vi "lab10.vi"() -> ()   [LabVIEW 2025]
uses:
  vi/thresholds.ctl
  vi/fpga_states.ctl
  <vilib>/rvi/Emulation/niFpgaGetClockAttributes.vi
  <vilib>/rvi/Emulation/niFpgaSctlEmulationGetInTimedLoop.vi
  <vilib>/rvi/Emulation/niFpgaEmulationReportErrorSimple.vi
  <vilib>/rvi/Emulation/niFpgaEmulationIsFPGAContextNoSignature.vi
  <vilib>/rvi/errors/niFpgaSetErrorForExecOnDevCompSimple.vi
  <vilib>/rvi/eio/common/nirviEmuReportErrorAndStop.vi
  <vilib>/rvi/DataTransferAndStorage/Container/Common/niFpgaContainerGetUniqueNameForEmu.vi
  <vilib>/rvi/FIFO/Fifo_Resource/nirvififoEmulationSetSize.vi
  <vilib>/rvi/FIFO/Fifo_Resource/nirviFifoEmulationQueueMgr.vi
  <instcachedir>/0/nirviFifoEmulationQueueMgr_E5CAEC123FF24DC58D834DCA3CDAA9B5.lvgen/nirviFifoEmulationQueueMgr_E5CAEC123FF24DC58D834DCA3CDAA9B5_002.vi
  <vilib>/Utility/error.llb/Clear Errors.vi
  <vilib>/rvi/FIFO/Fifo_Resource/nirvififoEmulationCreateLock.vi
  <vilib>/rvi/Emulation/niFpgaProcessEmulError.vi
  <vilib>/rvi/FIFO/Fifo_Resource/nirvififoEmulationObtainLock.vi
  <vilib>/rvi/FIFO/Fifo_Resource/nirvififoEmulationReleaseLock.vi
  <vilib>/rvi/occurrence/nirviWaitOnOccurrenceBase.vi
  <vilib>/rvi/errors/nirviReportUnexpectedCaseInternalError.vi
  <vilib>/rvi/errors/nirviReportUnexpectedCaseInternalError (U32).vi
  <vilib>/eio/utilities/niEioResolveVilibRelativePath.vi
  <vilib>/rvi/interface/RandomDataEmulation/niFpgaRandomDataHandleErrors.vi
  <vilib>/rvi/Emulation/niFpgaCriticalErrorInLSC.vi
  <instcachedir>/0/nirviFifoEmulationQueueMgr_E5CAEC123FF24DC58D834DCA3CDAA9B5.lvgen/nirviFifoEmulationQueueMgr_E5CAEC123FF24DC58D834DCA3CDAA9B5_003.vi
  <vilib>/rvi/FIFO/Fifo_Resource/nirvififoEmulationDetermineInputValidOut.vi
  <vilib>/rvi/eio/common/nirviEmuTemplateMethod_errors.vi
  <vilib>/rvi/Memory/Memory_Emulation/nirvimemoryFastEmulation.vi
  <vilib>/rvi/Memory/Memory_Emulation/nirvimemoryEmulation.vi
  <vilib>/rvi/DataTransferAndStorage/Container/Common/niFpgaContainerExecOnDevCompGetState.vi
  <vilib>/rvi/Memory/Memory_Emulation/niFpgaMemoryEmulationCacheClearOnFirstRun.vi
  <vilib>/rvi/Memory/Memory_Emulation/nirvimemoryEmulationManagerCache_MakeExclusive.vi
  <vilib>/rvi/Memory/Memory_Emulation/niFpgaMemoryEmulationValidateCache.vi
  <vilib>/rvi/Memory/Memory_Emulation/nirvimemoryEmulationManagerCache_InsertValue.vi
  <vilib>/rvi/Memory/Memory_Emulation/nirvimemoryEmulationManagerCache_ReleaseExclusive.vi
  <vilib>/rvi/Memory/Memory_Emulation/nirvimemoryEmulationManagerCache_GetValue.vi
  <vilib>/rvi/Memory/Memory_Emulation/nirvimemoryEmulationManagerCache_SetValue.vi
  <vilib>/rvi/Emulation/niFpgaSctlEmulationResourceMgr.vi
  <vilib>/rvi/DataTransferAndStorage/Container/XNode/niFpgaContainer.xnode
  <vilib>/rvi/FIFO/Fifo_Resource/nirvififoEmulationRead.vi
  <vilib>/rvi/interface/RandomDataEmulation/nirviRandomDataFpgaReadWriteTemplate.vi
  <vilib>/rvi/FIFO/Fifo_Resource/nirvififoEmulationWrite.vi
  <vilib>/eio/EIONode/EIONode.xnode
  <vilib>/rvi/Memory/Memory_Emulation/niFpgaMemoryEmulationRefIn.vi
panel:
  in  "Threshold":T1
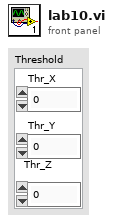
[diagram p1: front panel]
types:
  T1 = typedef "thresholds.ctl" = cluster{"Thr_X":i16, "Thr_Y":i16, "Thr_Z":i16}
  T2 = typedef "fpga_states.ctl" = enum16{"Wait", "Collect"}
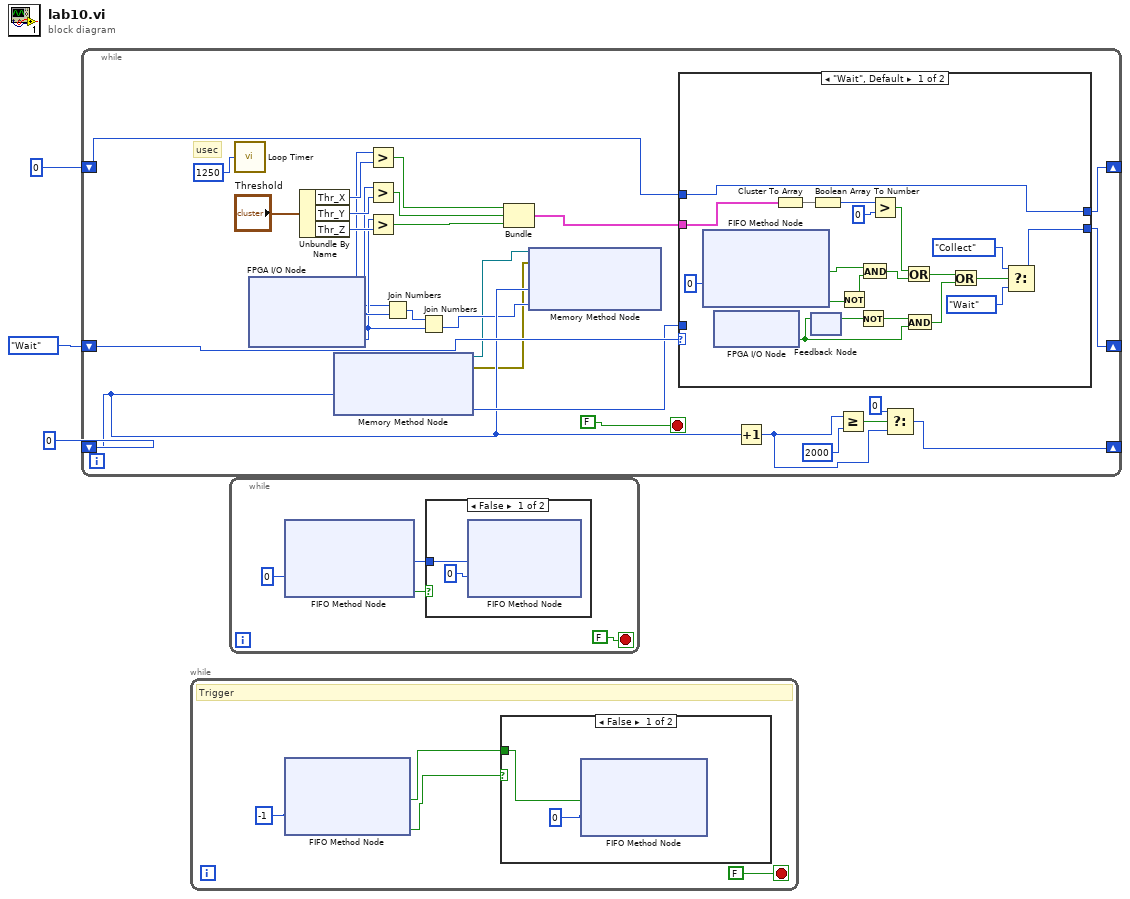
[diagram p0: block diagram]
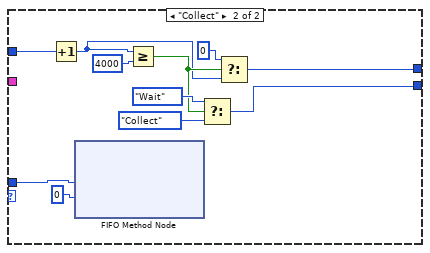
[diagram p4: hidden frame]
diagram:
  n1 = while {
    shift-right: [w28] -> _
    shift-left: i16 0 -> [w29]
    shift-right: [w18] -> _
    shift-left: fpga_states."Wait" -> [w19]
    shift-right: [w9] -> _
    shift-left: u32 0 -> [w7]
    stop <- FALSE stop-if-true
    # "usec"
    n2 = call "Loop Timer"("Count(uSec)"=u32 1250) -> ()  [unwired: 1 out]
    n3 = xnode "FPGA I/O Node"() -> ("AccelerationX"=w14:i16, "AccelerationY"=w16:i16, "AccelerationZ"=w15:i16)  [unwired: 3 in, 3 out]
    n4 = Unbundle By Name("Threshold") -> ("Thr_X"=w26:i16, "Thr_Y"=w25:i16, "Thr_Z"=w24:i16)
    n5 = xnode ("Memory Method Node")("Address"=w7) -> ("Data"=w8:u64, "error out"=w4:errorcluster, "Memory Out"=w5:refnum<k21>)  [unwired: 2 in]
    n6 = Greater?(x=w14, y=w26) -> (0:w23:bool)
    n7 = Greater?(x=w16, y=w25) -> (0:w22:bool)
    n8 = Greater?(x=w15, y=w24) -> (0:w21:bool)
    n9 = Join Numbers(hi=w14, lo=w16) -> ((hi.lo)=w17:u32)
    n10 = Join Numbers(hi=w17, lo=w15) -> ((hi.lo)=w6:u64)
    n11 = Bundle(w23, w22, w21) -> (w20:cluster{bool, bool, bool})  [unwired: 1 in]
    n12 = xnode ("Memory Method Node")("Address"=w7, "Data"=w6, "error in (no error)"=w4, "Memory In"=w5) -> ()  [unwired: 2 out]
    n13 = case shown="\"Wait\", Default" w19 {
      tunnel: w29 -> [w49 w55]
      tunnel: [w49 w54] -> w28
      tunnel: w20 -> [w51 _]
      tunnel: [w44 w53] -> w18
      tunnel: w8 -> [_ w52]
      frame "Wait", Default {
        n14 = xnode ("FIFO Method Node")("Timeout"=0) -> ("Element"=w34:bool, "Timed Out?"=w35:bool)  [unwired: 1 in, 1 out]
        n15 = xnode "FPGA I/O Node"() -> ("Button0"=w40:bool)  [unwired: 1 in, 1 out]
        n16 = Cluster To Array(cluster=w51) -> (array=w50:bool[])
        n17 = feedback-in #1(w40) -> ()
        n18 = feedback #1() -> (w38:bool)  [unwired: 1 in]
        n19 = Boolean Array To Number(Boolean array=w50) -> (number=w48:u8)
        n20 = Not(x=w35) -> (.not. x?=w33:bool)
        n21 = Not(x=w38) -> (.not. x?=w39:bool)
        n22 = And(x=w34, y=w33) -> (x .and. y?=w32:bool)
        n23 = Greater?(x=w48, y=u8 0) -> (0:w43:bool)
        n24 = Or(x=w43, y=w32) -> (x .or. y?=w42:bool)
        n25 = And(x=w39, y=w40) -> (x .and. y?=w37:bool)
        n26 = Or(x=w42, y=w37) -> (x .or. y?=w41:bool)
        n27 = Select(t=fpga_states."Collect", s=w41, f=fpga_states."Wait") -> (s? t:f=w44:T2)
      }
      frame "Collect" {
        n28 = Increment(x=w55) -> (x+1=w57:i16)
        n29 = xnode ("FIFO Method Node")("Element"=w52, "Timeout"=0) -> ()  [unwired: 1 in, 2 out]
        n30 = Greater Or Equal?(x=w57, y=i16 4000) -> (x >= y?=w58:bool)
        n31 = Select(t=fpga_states."Wait", s=w58, f=fpga_states."Collect") -> (s? t:f=w53:T2)
        n32 = Select(t=i16 0, s=w58, f=w57) -> (s? t:f=w54:i16)
      }
    }
    n33 = Increment(x=w7) -> (x+1=w11:u32)
    n34 = Greater Or Equal?(x=w11, y=u32 2000) -> (x >= y?=w12:bool)
    n35 = Select(t=u32 0, s=w12, f=w11) -> (s? t:f=w9:u32)
  }
  n36 = while {
    stop <- FALSE stop-if-true
    # "Trigger"
    n37 = xnode ("FIFO Method Node")("Timeout"=-1) -> ("Element"=w64:bool, "Timed Out?"=w63:bool)  [unwired: 1 in, 1 out]
    n38 = case shown="False" w63 {
      tunnel: w64 -> [w68 _]
      frame False {
        n39 = xnode ("FIFO Method Node")("Element"=w68, "Timeout"=0) -> ()  [unwired: 1 in, 2 out]
      }
      frame True {
      }
    }
  }
  n40 = while {
    stop <- FALSE stop-if-true
    n41 = xnode ("FIFO Method Node")("Timeout"=0) -> ("Element"=w71:u64, "Timed Out?"=w72:bool)  [unwired: 1 in, 1 out]
    n42 = case shown="False" w72 {
      tunnel: w71 -> [w73 _]
      frame False {
        n43 = xnode ("FIFO Method Node")("Element"=w73, "Timeout"=0) -> ()  [unwired: 1 in, 2 out]
      }
      frame True {
      }
    }
  }
